vi "file.open.vi"(8 "error in":errorcluster, 11 "Path to MIDI File (use dialog)":path) -> (0 "error out":errorcluster, 2 "Path to MIDI File":path, 3 "midi-file out":refnum<class "midi-file.lvclass">)   [LabVIEW 2020, in "midi-file.lvclass"]
uses:
  midi-file.lvclass
  midi-file.lvclass/midi-file.ctl
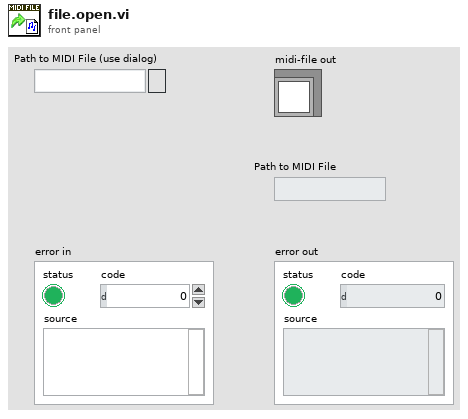
[diagram p1: front panel]
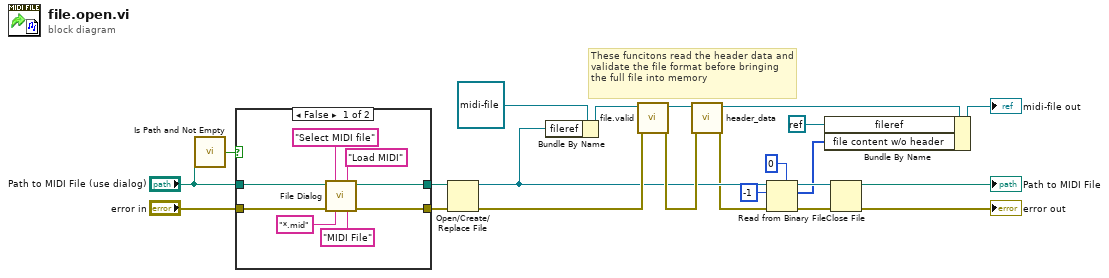
[diagram p0: block diagram]
diagram:
  # "These funcitons read the header data and validate the file format before bringing the full file into memory"
  n1 = call <vilib>:"Is Path and Not Empty.vi"("path"="Path to MIDI File (use dialog)") -> ("Is Path and Not Empty?"=w6:bool)  [unwired: 4 in]
  n2 = case shown="False" w6 {
    tunnel: [w25 w32] -> w5
    tunnel: "error in" -> [w24 w32]
    tunnel: "Path to MIDI File (use dialog)" -> [w27 w31]
    tunnel: [w26 w31] -> w2
    frame False {
      n3 = call "File Dialog"("start path"=w27, "prompt"="Select MIDI file", "button label"="Load MIDI", "error in"=w24, "pattern (all files)"="*.mid", "pattern label"="MIDI File") -> ("selected path"=w26:path, "error out"=w25:errorcluster)  [unwired: 6 in, 2 out]
    }
    frame True {
    }
  }
  n4 = Open/Create/Replace File(file path (use dialog)=w2, error in=w5) -> (refnum out=w17:refnum<file>, error out=w20:errorcluster)  [unwired: 4 in, 1 out]
  n5 = Bundle By Name(cluster=refnum<class "midi-file.lvclass"> refnum ("midi-file out"), "fileref"=w17) -> (w21:refnum<class "midi-file.lvclass">)
  n6 = call "file.valid.vi"("error in"=w20, "midi-file in"=w21) -> ("error out"=w18:errorcluster, "midi-file out"=w19:refnum<class "midi-file.lvclass">)  [unwired: 8 in]
  n7 = call "header_data.vi"("error in"=w18, "midi-file in"=w19) -> ("error out"=w12:errorcluster, "midi-file out"=w10:refnum<class "midi-file.lvclass">)  [unwired: 8 in]
  n8 = Read from Binary File(5:u8 0, 8:w12, 10:-1 ("count (1)"), 11:w17) -> (0:w13:errorcluster, 2:w8:u8[], 3:w14:refnum<file>)  [unwired: 2 in, 1 out]
  n9 = Bundle By Name(cluster=w10, "fileref"=refnum<k0> refnum, "file content w/o header"=w8) -> (→"midi-file out":refnum<class "midi-file.lvclass">)
  n10 = Close File(refnum=w14, error in=w13) -> (path=→"Path to MIDI File":path, error out=→"error out":errorcluster)
